vi "DSS-Tests-data_path.vi"(11 "relative path":string) -> (3 "path":path)   [LabVIEW 2020, in "DSS-Tests.lvlib"]
doc: "Builds the absolute path of a test data file from its path relative to the repository root, written with forward slashes (e.g. data/calibration-standards/sim-P1-open.s2p)."
uses:
  DSS-Tests.lvlib
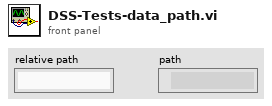
[diagram p1: front panel]
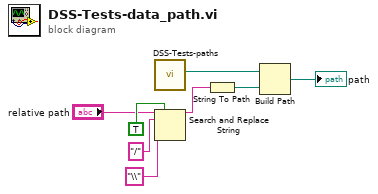
[diagram p0: block diagram]
diagram:
  n1 = call "DSS-Tests-paths.vi"() -> ("repo root"=w2:path)  [unwired: 10 in, 1 out]
  n2 = Search and Replace String(replace all?=TRUE ("replace all"), input string="relative path", search string="/" ("slash"), replace string="\\" ("backslash")) -> (result string=w6:string)  [unwired: 4 in, 3 out]
  n3 = String To Path(string=w6) -> (path=w7:path)
  n4 = Build Path(base path=w2, name or relative path=w7) -> (appended path=→"path":path)
